vi "Delete In Folder.vi"(8 "error in (no error)":errorcluster, 10 "ProjectItem in":refnum<vi>) -> (0 "error out":errorcluster)   [LabVIEW 2019, in "gRPC Template Creation Utility.lvlib"]
uses:
  gRPC Template Creation Utility.lvlib
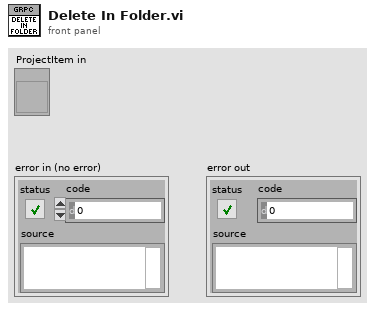
[diagram p1: front panel]
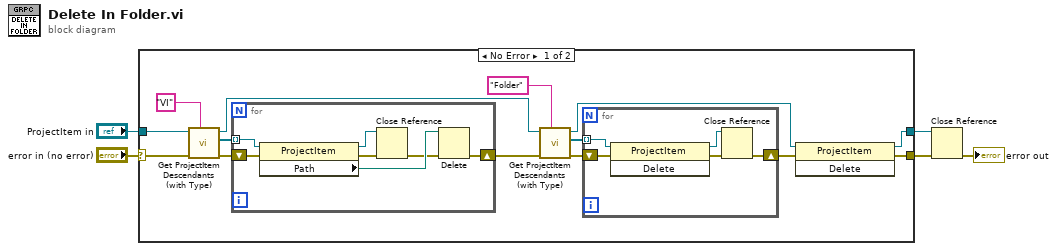
[diagram p0: block diagram]
diagram:
  n1 = case shown="No Error" "error in (no error)" {
    selector: "error in (no error)" -> [w9 w33]
    tunnel: "ProjectItem in" -> [w19 w32]
    tunnel: [w6 w33] -> w1
    tunnel: [w7 w32] -> w3
    frame No Error {
      n2 = call "Get ProjectItem Descendants (with Type).vi"("Type"="VI", "error in (no error)"=w9, "ProjectItem in"=w19) -> ("error out"=w8:errorcluster, "All Descendents"=w17:refnum<vi>[], "ProjectItem out"=w16:refnum<vi>)  [unwired: 6 in]
      n3 = for {
        tunnel: w17 -> [w31] mode=indexing
        shift-right: [w25] -> w13
        shift-left: w8 -> [w28]
        n4 = property class="ProjectItem"(reference=w31, error in=w28) -> (reference out=w30:refnum<vi>, error out=w27:errorcluster, "Path"=w29:path)
        n5 = Close Reference(reference=w30, error in (no error)=w27) -> (error out=w26:errorcluster)
        n6 = Delete(path (use dialog)=w29, error in=w26) -> (error out=w25:errorcluster)  [unwired: 3 in, 2 out]
      }
      n7 = call "Get ProjectItem Descendants (with Type).vi"("Type"="Folder", "error in (no error)"=w13, "ProjectItem in"=w16) -> ("error out"=w12:errorcluster, "All Descendents"=w14:refnum<vi>[], "ProjectItem out"=w11:refnum<vi>)  [unwired: 6 in]
      n8 = for {
        tunnel: w14 -> [w24] mode=indexing
        shift-right: [w20] -> w10
        shift-left: w12 -> [w22]
        n9 = invoke class="ProjectItem" method="Delete"(reference=w24, error in=w22) -> (reference out=w23:refnum<vi>, error out=w21:errorcluster)  [unwired: 1 in, 1 out]
        n10 = Close Reference(reference=w23, error in (no error)=w21) -> (error out=w20:errorcluster)
      }
      n11 = invoke class="ProjectItem" method="Delete"(reference=w11, error in=w10) -> (reference out=w7:refnum<vi>, error out=w6:errorcluster)  [unwired: 1 in, 1 out]
    }
    frame Error {
    }
  }
  n12 = Close Reference(reference=w3, error in (no error)=w1) -> (error out=→"error out":errorcluster)
